vi "Unpack Actor Data Msg.vi"(11 "Actor Data Msg":refnum<class "Observe Data Msg.lvclass">) -> (1 "Publication Time":timestamp, 2 "Value":variant, 3 "Datum Name":string)   [LabVIEW 2018, in "MVA Framework.lvlib" / "IObserver.lvlib" / "Observe Data Msg.lvclass"]
doc: "解包操作者数据消息"
uses:
  Observe Data Msg.lvclass
  Observe Data Msg.lvclass/Observe Data Msg.ctl
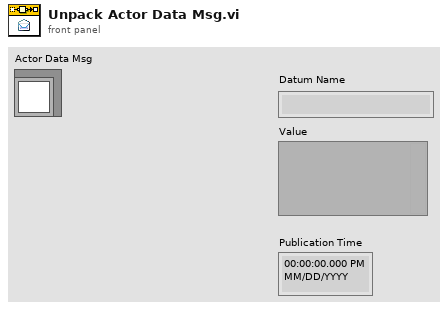
[diagram p1: front panel]
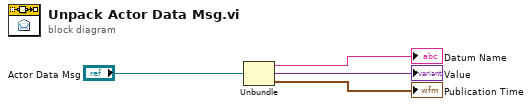
[diagram p0: block diagram]
diagram:
  n1 = Unbundle("Actor Data Msg") -> (→"Datum Name":string, →"Value":variant, →"Publication Time":timestamp)
